vi "test modern missing meta.vi"(8 "error in (no error)":errorcluster) -> (0 "error out":errorcluster, 3 "body":string)   [LabVIEW 2020, in "MCP Server tests.lvlib"]
doc: "A request that is modern by its MCP-Protocol-Version header (or by being server/discover) must carry params._meta with io.modelcontextprotocol/protocolVersion. Without _meta and with _meta lacking the protocolVersion it is answered HTTP 400 with the JSON-RPC error -32602 and the request id echoed - also tools/list, which before was routed to the legacy era and answered 200. The requests are sent with the LabVIEW HTTP Client directly."
uses:
  MCP Server tests.lvlib
  <vilib>/addons/_JKI Toolkits/Caraya/classes/Test/Test.lvclass
  <vilib>/addons/_JKI Toolkits/Caraya/classes/Assert/Assert.lvclass
panel:
  out "lookup error":errorcluster
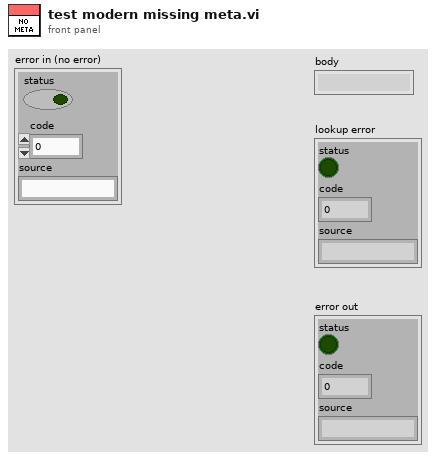
[diagram p1: front panel]
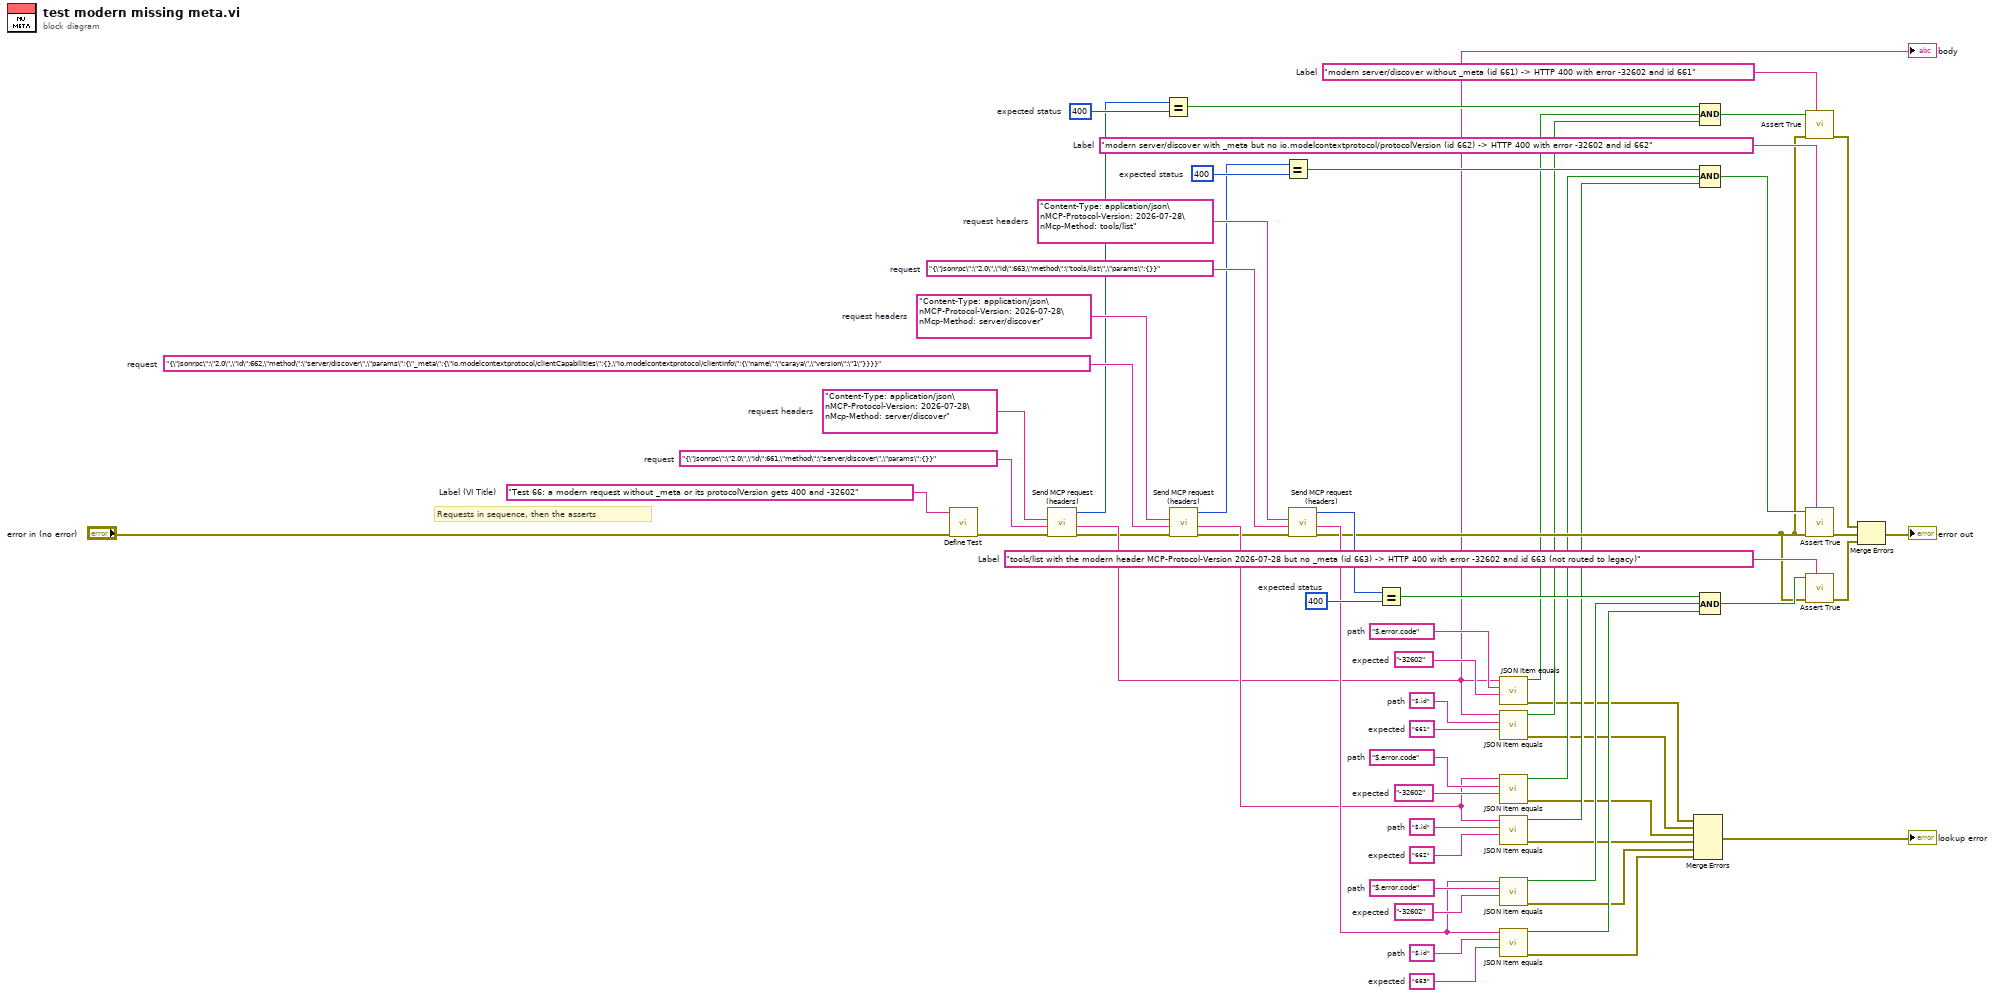
[diagram p0: block diagram]
diagram:
  w57 = "tools/list with the modern header MCP-Protocol-Version 2026-07-28 but no _meta (id 663) -> HTTP 400 with error -32602 and id 663 (not routed to legacy)"  # Label
  w54 = "modern server/discover with _meta but no io.modelcontextprotocol/protocolVersion (id 662) -> HTTP 400 with error -32602 and id 662"  # Label
  w51 = "modern server/discover without _meta (id 661) -> HTTP 400 with error -32602 and id 661"  # Label
  w46 = "663"  # expected
  w45 = "$.id"  # path
  w42 = "-32602"  # expected
  w41 = "$.error.code"  # path
  w39 = 400  # expected status
  w35 = "Content-Type: application/json\nMCP-Protocol-Version: 2026-07-28\nMcp-Method: tools/list"  # request headers
  w34 = "{\"jsonrpc\":\"2.0\",\"id\":663,\"method\":\"tools/list\",\"params\":{}}"  # request
  w31 = "662"  # expected
  w30 = "$.id"  # path
  w27 = "-32602"  # expected
  w26 = "$.error.code"  # path
  w24 = 400  # expected status
  w20 = "Content-Type: application/json\nMCP-Protocol-Version: 2026-07-28\nMcp-Method: server/discover"  # request headers
  w19 = "{\"jsonrpc\":\"2.0\",\"id\":662,\"method\":\"server/discover\",\"params\":{\"_meta\":{\"io.modelcontextprotocol/clientCapabilities\":{},\"io.modelcontextprotocol/clientInfo\":{\"name\":\"caraya\",\"version\":\"1\"}}}}"  # request
  w16 = "661"  # expected
  w15 = "$.id"  # path
  w12 = "-32602"  # expected
  w11 = "$.error.code"  # path
  w9 = 400  # expected status
  w5 = "Content-Type: application/json\nMCP-Protocol-Version: 2026-07-28\nMcp-Method: server/discover"  # request headers
  w4 = "{\"jsonrpc\":\"2.0\",\"id\":661,\"method\":\"server/discover\",\"params\":{}}"  # request
  w2 = "Test 66: a modern request without _meta or its protocolVersion gets 400 and -32602"  # Label (VI Title)
  # "Requests in sequence, then the asserts"
  n1 = call <vilib>:"Define Test.vi"("error in (no error)"="error in (no error)", "Label (VI Title)"=w2) -> ("error out"=w3:errorcluster)  [unwired: 8 in, 1 out]
  n2 = call "Send MCP request (headers).vi"("error in (no error)"=w3, "request"=w4, "request headers"=w5) -> ("error out"=w6:errorcluster, "response"=w7:string, "status code"=w8:i32)  [unwired: 5 in, 1 out]
  "body" <- w7
  n3 = Equal?(x=w8, y=w9) -> (x = y?=w10:bool)
  n4 = call "Send MCP request (headers).vi"("error in (no error)"=w6, "request"=w19, "request headers"=w20) -> ("error out"=w21:errorcluster, "response"=w22:string, "status code"=w23:i32)  [unwired: 5 in, 1 out]
  n5 = Equal?(x=w23, y=w24) -> (x = y?=w25:bool)
  n6 = call "Send MCP request (headers).vi"("error in (no error)"=w21, "request"=w34, "request headers"=w35) -> ("error out"=w36:errorcluster, "response"=w37:string, "status code"=w38:i32)  [unwired: 5 in, 1 out]
  n7 = Equal?(x=w38, y=w39) -> (x = y?=w40:bool)
  n8 = call "JSON item equals.vi"("expected"=w12, "path"=w11, "JSON"=w7) -> ("error out"=w13:errorcluster, "equal?"=w14:bool)  [unwired: 6 in, 1 out]
  n9 = call "JSON item equals.vi"("expected"=w16, "path"=w15, "JSON"=w7) -> ("error out"=w17:errorcluster, "equal?"=w18:bool)  [unwired: 6 in, 1 out]
  n10 = call "JSON item equals.vi"("expected"=w27, "path"=w26, "JSON"=w22) -> ("error out"=w28:errorcluster, "equal?"=w29:bool)  [unwired: 6 in, 1 out]
  n11 = call "JSON item equals.vi"("expected"=w31, "path"=w30, "JSON"=w22) -> ("error out"=w32:errorcluster, "equal?"=w33:bool)  [unwired: 6 in, 1 out]
  n12 = call "JSON item equals.vi"("expected"=w42, "path"=w41, "JSON"=w37) -> ("error out"=w43:errorcluster, "equal?"=w44:bool)  [unwired: 6 in, 1 out]
  n13 = call "JSON item equals.vi"("expected"=w46, "path"=w45, "JSON"=w37) -> ("error out"=w47:errorcluster, "equal?"=w48:bool)  [unwired: 6 in, 1 out]
  n14 = Merge Errors(w13, w17, w28, w32, w43, w47) -> (→"lookup error":errorcluster)
  n15 = Compound Arithmetic op=AND(w10, w14, w18) -> (w50:bool)
  n16 = Compound Arithmetic op=AND(w25, w29, w33) -> (w53:bool)
  n17 = Compound Arithmetic op=AND(w40, w44, w48) -> (w56:bool)
  n18 = call <vilib>:"Assert True.vi"("Label"=w51, "error in (no error)"=w36, "True?"=w50) -> ("error out"=w52:errorcluster)  [unwired: 7 in, 1 out]
  n19 = call <vilib>:"Assert True.vi"("Label"=w54, "error in (no error)"=w36, "True?"=w53) -> ("error out"=w55:errorcluster)  [unwired: 7 in, 1 out]
  n20 = call <vilib>:"Assert True.vi"("Label"=w57, "error in (no error)"=w36, "True?"=w56) -> ("error out"=w58:errorcluster)  [unwired: 7 in, 1 out]
  n21 = Merge Errors(w52, w55, w58) -> (→"error out":errorcluster)
